vi "Read Loop.vi"(8 "error in (no error)":errorcluster caption="에러 입력(에러 없음)", 11 "TCP Socket 입력":refnum<class "TCP Socket.lvclass">) -> (0 "error out":errorcluster caption="에러 출력", 3 "TCP Socket 출력":refnum<class "TCP Socket.lvclass">)   [LabVIEW 2023, in "TCP Socket.lvclass"]
uses:
  TCP Socket.lvclass
  TCP Socket.lvclass/TCP Socket.ctl
panel:
  out "값":u32
  out "데이터 출력 2":string
  out "데이터 출력":string
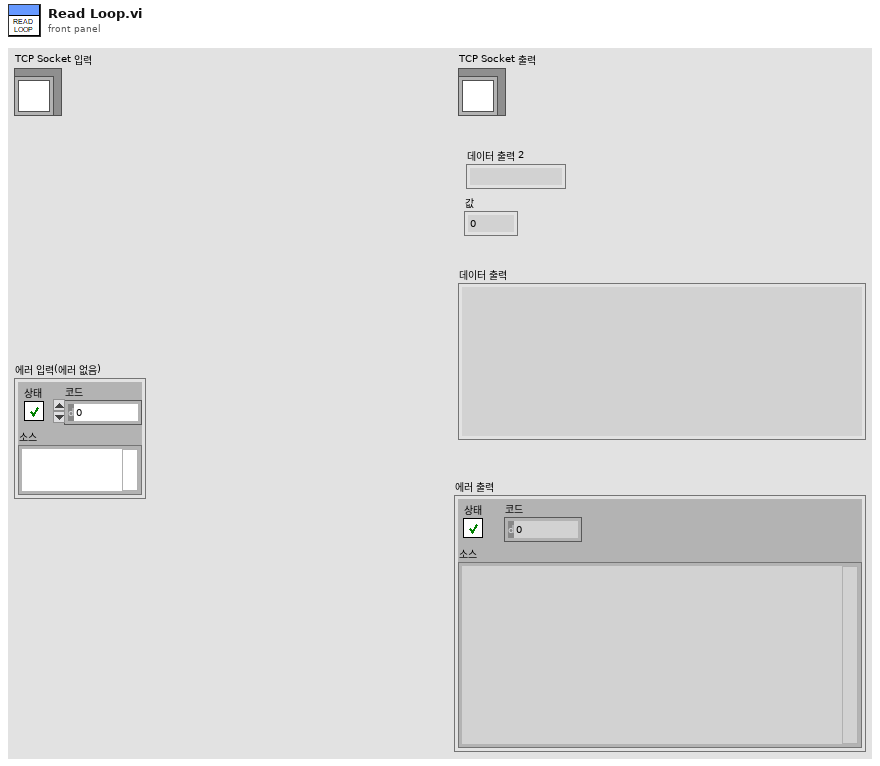
[diagram p1: front panel]
types:
  T1 = enum16{"big-endian, network order", "native, host order", "little-endian"}
  T2 = cluster{"Reader Q":refnum<queue>, "Writer Q":refnum<queue>}
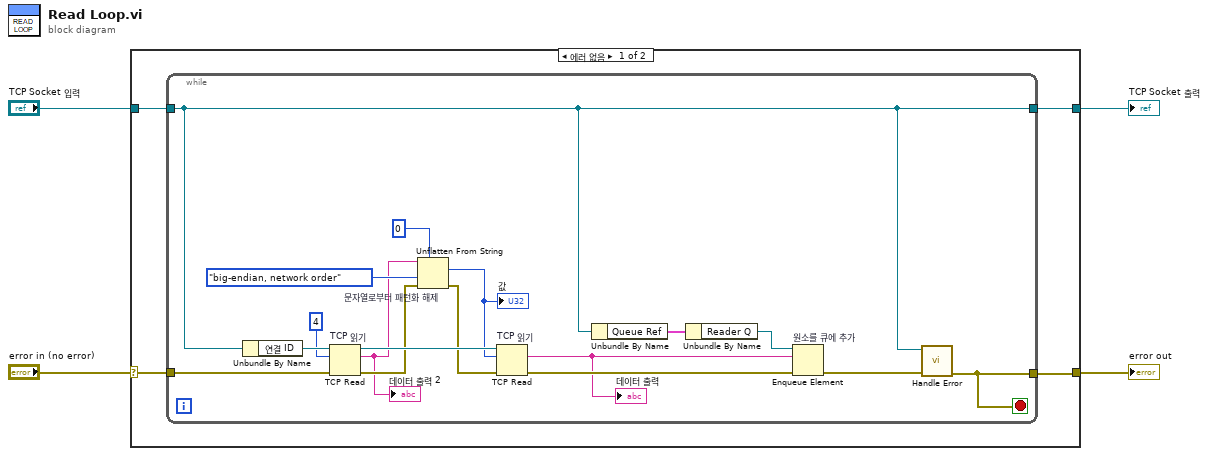
[diagram p0: block diagram]
diagram:
  n1 = case shown="에러 없음" "error in (no error)" {
    selector: "error in (no error)" -> [w6 w27]
    tunnel: [w5 w27] -> w3
    tunnel: [w7 w26] -> w1
    tunnel: "TCP Socket 입력" -> [w8 w26]
    frame No Error {
      n2 = while {
        tunnel: w8 -> [w17]
        tunnel: [w17] -> w7
        tunnel: w6 -> [w22]
        tunnel: [w18] -> w5
        stop <- w18 stop-if-true
        n3 = Unbundle By Name(w17) -> ("연결 ID"=w23:refnum<k5>)
        n4 = TCP Read "TCP 읽기"(connection ID=w23, bytes to read=4 ("읽을 바이트"), error in (no error)=w22) -> (connection ID out=w24:refnum<k5>, data out=w10:string, error out=w13:errorcluster)  [unwired: 2 in]
        "데이터 출력 2" <- w10
        n5 = Unflatten From String "문자열로부터 패턴화 해제"(type=u32 0, binary string=w10, byte order (0:big-endian, network order)=T1."big-endian, network order" ("바이트 순서(0:big-endian, network order)"), error in (no error)=w13) -> (value=w9:u32, error out=w12:errorcluster)  [unwired: 1 in, 1 out]
        "값" <- w9
        n6 = TCP Read "TCP 읽기"(connection ID=w24, bytes to read=w9, error in (no error)=w12) -> (data out=w11:string, error out=w25:errorcluster)  [unwired: 2 in, 1 out]
        "데이터 출력" <- w11
        n7 = Unbundle By Name(w17) -> ("Queue Ref"=w21:T2)
        n8 = Unbundle By Name(w21) -> ("Reader Q"=w20:refnum<queue>)
        n9 = Enqueue Element "원소를 큐에 추가"(queue=w20, element=w11, error in (no error)=w25) -> (error out=w19:errorcluster)  [unwired: 1 in, 2 out]
        n10 = call "Handle Error.vi"("error in (no error)"=w19, "TCP Socket 입력"=w17) -> ("error out"=w18:errorcluster)  [unwired: 8 in, 1 out]
      }
    }
    frame Error {
    }
  }
  "error out" <- w3
  "TCP Socket 출력" <- w1
